vi "serialization tests.vi"() -> (0 "no error":errorcluster, 3 "channels equal":bool)   [LabVIEW 2013, in "CVT tests.lvlib"]
uses:
  CVT tests.lvlib
  <vilib>/NI/Tag Bus Module Framework/channel/channel classification.ctl
  configuration/CVT configuration.lvclass
  configuration/CVT configuration.lvclass/CVT configuration.ctl
  configuration/Write channels.vi
  configuration/Read channels.vi
  <vilib>/NI/Tag Bus Module Framework/channel/TBM channel.lvclass
  <vilib>/NI/Configuration Framework/serializable configuration/NISE_CEF_serializable configuration.lvclass
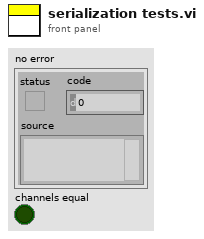
[diagram p1: front panel]
types:
  T1 = typedef "TBM channel.lvclass/channel classification.ctl" = enum16{"input data", "output data", "processing parameter", "processing result"}
  T2 = typedef "tag bus.lvlib/tag descriptor.lvclass/Data Type.ctl" = enum16{"Double", "Single", "I64", "I32", "I16", "I8", "U64", "U32", "U16", "U8", "Boolean", "String", "Array of Double", "Array of Single", "Array of I64", "Array of I32", "Array of I16", "Array of I8", "Array of U64", "Array of U32", "Array of U16", "Array of U8", "Array of Boolean", "Array of String"}
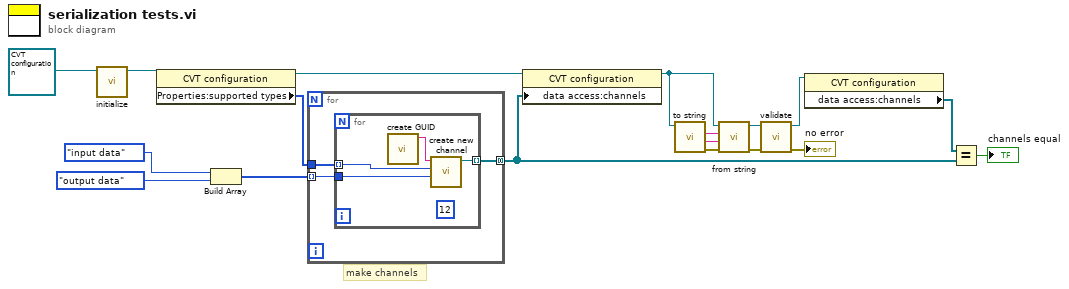
[diagram p0: block diagram]
diagram:
  # "make channels"
  n1 = call <vilib>:"initialize.vi"("configuration in"=refnum<class "CVT configuration.lvclass"> refnum ("tag bus configurable plugin module configuration")) -> ("configuration out"=w1:refnum<class "CVT configuration.lvclass">)  [unwired: 8 in, 2 out]
  n2 = property class="CVT configuration"(reference=w1) -> (reference out=w7:refnum<class "CVT configuration.lvclass">, "Properties:supported types"=w10:T2[])  [unwired: 1 in, 1 out]
  n3 = Build Array(channel_classification."input data" ("channel classification"), channel_classification."output data" ("channel classification")) -> (w11:T1[])
  n4 = for {
    tunnel: w11 -> [w21] mode=indexing
    tunnel: [w20] -> w3 mode=concatenating
    tunnel: w10 -> [w19]
    n5 = for {
      tunnel: w21 -> [w24]
      tunnel: [w25] -> w20 mode=indexing
      tunnel: w19 -> [w23] mode=indexing
      (unwired) 12
      n6 = call <vilib>:"create GUID.vi"() -> ("uuid"=w22:string)  [unwired: 10 in, 1 out]
      n7 = call <vilib>:"create new channel.vi"("channel classification"=w24, "data type"=w23, "channel name"=w22) -> ("channel"=w25:refnum<class "TBM channel.lvclass">)  [unwired: 8 in]
    }
  }
  n8 = property class="CVT configuration"(reference=w7, "data access:channels"=w3) -> (reference out=w4:refnum<class "CVT configuration.lvclass">)  [unwired: 1 in, 1 out]
  n9 = call-dynamic "to string.vi"("CVT configuration in"=w4) -> ("error out"=w18:errorcluster, "data"=w17:string, "version"=w16:string)  [unwired: 7 in, 1 out]
  n10 = call-dynamic "from string.vi"("error in"=w18, "data"=w17, "version"=w16, "CVT configuration in"=w4) -> ("error out"=w9:errorcluster, "CVT configuration out"=w15:refnum<class "CVT configuration.lvclass">)  [unwired: 6 in]
  n11 = call-dynamic "validate.vi"("error in"=w9, "CVT configuration in"=w15) -> ("error out"=→"no error":errorcluster, "CVT configuration out"=w6:refnum<class "CVT configuration.lvclass">)  [unwired: 8 in]
  n12 = property class="CVT configuration"(reference=w6) -> ("data access:channels"=w5:refnum<class "TBM channel.lvclass">[])  [unwired: 1 in, 2 out]
  n13 = Equal?(x=w5, y=w3) -> (x = y?=→"channels equal":bool)
